vi "Start Entry.vi"(4 "Project Store in":refnum<class "Project Store.lvclass">, 6 "Start Time":timestamp, 7 "Time Entry Store in":refnum<class "Time Entry Store.lvclass">, 8 "error in":errorcluster, 9 "Description":string, 10 "Task ID":string, 11 "Project ID":string) -> (0 "error out":errorcluster, 3 "New Entry":T1, 5 "Time Entry Store out":refnum<class "Time Entry Store.lvclass">)   [LabVIEW 2026]
doc: "Starts a new time entry: gives it a new ID (Time Entry Store New Time Entry) and saves it with End Time 0, which marks it as running. When Project ID or Task ID is empty nothing is saved and error 5101 is returned (Start Entry: select a project and a task first.); New Entry then carries the inputs with an empty ID.\n\nInputs: Project ID; Task ID; Description; Start Time; Time Entry Store in; Project Store in (optional, supplies the project and task name labels written to the file); error in.\nOutputs: New Entry; Time Entry Store out; error out.\n\nGenerated by: Claude"
uses:
  Storage/Time Entry Store/Time Entry Store.lvclass
  Storage/Project Store/Project Store.lvclass
  Storage/Rows/Time Entry.ctl
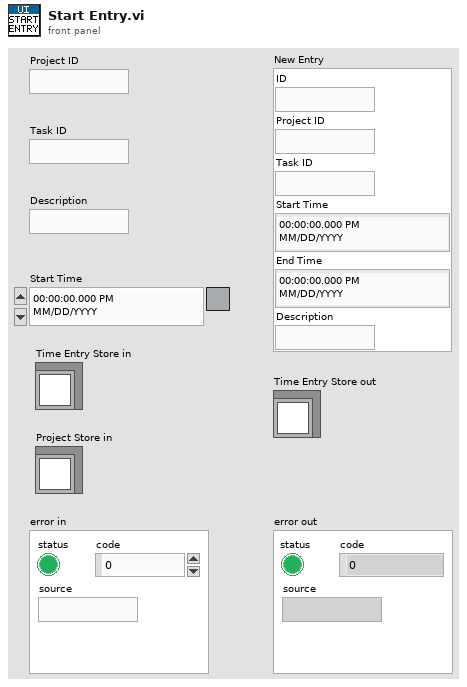
[diagram p1: front panel]
types:
  T1 = typedef "Time Entry.ctl" = cluster{"ID":string, "Project ID":string, "Task ID":string, "Start Time":timestamp, "End Time":timestamp, "Description":string}
  T2 = cluster{"ID":string, "Project ID":string, "Task ID":string, "Start Time":timestamp, "End Time":timestamp, "Description":string}
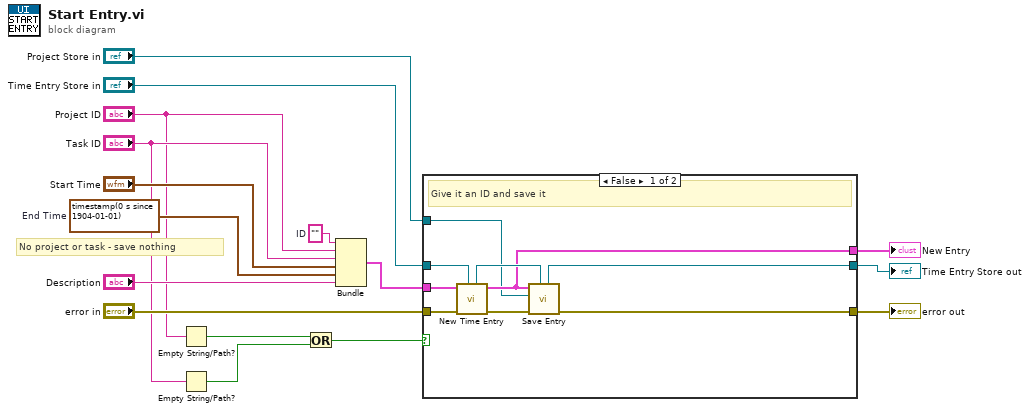
[diagram p0: block diagram]
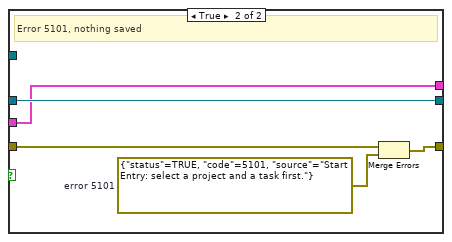
[diagram p2: hidden frame]
diagram:
  w12 = timestamp(0 s since 1904-01-01)  # End Time
  w11 = ""  # ID
  # "No project or task - save nothing"
  n1 = Empty String/Path?(string/path="Project ID") -> (empty?=w14:bool)
  n2 = Empty String/Path?(string/path="Task ID") -> (empty?=w15:bool)
  n3 = Or(x=w14, y=w15) -> (x .or. y?=w16:bool)
  n4 = Bundle("ID"=w11, "Project ID"="Project ID", "Task ID"="Task ID", "Start Time"="Start Time", "End Time"=w12, "Description"="Description") -> (w13:T2)  [unwired: 1 in]
  n5 = case shown="False" w16 {
    tunnel: "Time Entry Store in" -> [w18 w27]
    tunnel: "Project Store in" -> [w19 _]
    tunnel: "error in" -> [w20 w28]
    tunnel: w13 -> [w17 w26]
    tunnel: [w21 w26] -> w8
    tunnel: [w24 w27] -> w9
    tunnel: [w25 w30] -> w10
    frame False {
      # "Give it an ID and save it"
      n6 = call "New Time Entry.vi"("Time Entry Store in"=w18, "error in (no error)"=w20, "Time Entry"=w17) -> ("error out"=w23:errorcluster, "New Time Entry"=w21:T1, "Time Entry Store out"=w22:refnum<class "Time Entry Store.lvclass">)  [unwired: 6 in]
      n7 = call-dynamic "Save Entry.vi"("Time Entry Store in"=w22, "error in (no error)"=w23, "Project Store"=w19, "Time Entry"=w21) -> ("error out"=w25:errorcluster, "Time Entry Store out"=w24:refnum<class "Time Entry Store.lvclass">)  [unwired: 6 in]
    }
    frame True {
      w29 = errorcluster {"status"=TRUE, "code"=5101, "source"="Start Entry: select a project and a task first."}  # error 5101
      # "Error 5101, nothing saved"
      n8 = Merge Errors(w28, w29) -> (w30:errorcluster)
    }
  }
  "New Entry" <- w8
  "Time Entry Store out" <- w9
  "error out" <- w10
